vi "New Basic Scope.vi"   [LabVIEW 2018, in "GLog.lvlib" / "Basic.lvclass"]
doc: "Create a new Scope which filters log calls based on their Call Chain. Use this VI to configure a logger to only capture log calls only from within a specific Library, Class, or VI's call chain.\nFor example:\nIf \"A.vi\" calls \"B.vi\" and \"C.vi\", and \"B.vi\" also calls \"C.vi\", a Scope can ensure a logger only processes log calls from \"C.vi\" when it is called from \"B.vi\" and is ignored if it is called from \"A.vi\"."
uses:
  Basic.lvclass
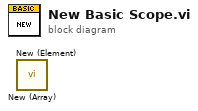
[diagram p0: block diagram]
diagram:
  n1 = call "New (Array).vi"() -> ()  [unwired: 11 in, 1 out]
  n2 = call "New (Element).vi"() -> ()  [unwired: 11 in, 1 out]
